vi "GetUserModePrefPath.vi"(8 "error in (no error)":errorcluster) -> (3 "prefpath":path)   [LabVIEW 2023]
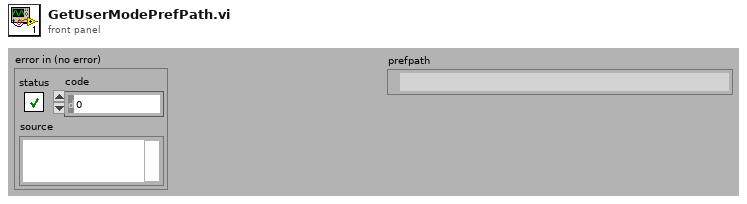
[diagram p1: front panel]
types:
  T1 = enum32{"invalid CPU target", "Motorola 68K", "PowerPC", "Intel x86", "SPARC", "PA-RISC", "MIPS", "Alpha", "ARM", "AMD/Intel x64", "ARM64"}
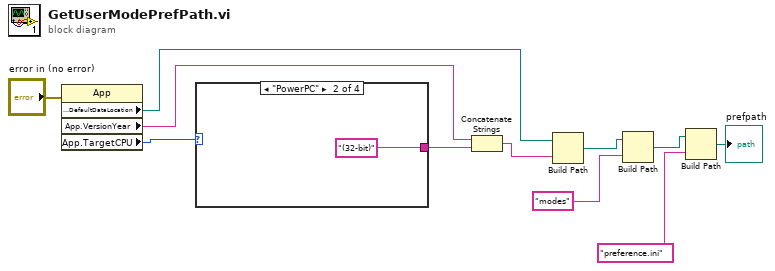
[diagram p0: block diagram]
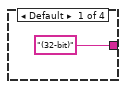
[diagram p2: hidden frame]
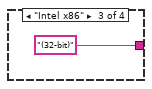
[diagram p3: hidden frame]
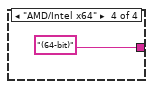
[diagram p4: hidden frame]
diagram:
  n1 = property class="App"(error in="error in (no error)") -> ("App.DefaultDataLocation"=w8:path, "App.VersionYear"=w9:string, "App.TargetCPU"=w11:T1)  [unwired: 1 in, 2 out]
  n2 = case shown="\"PowerPC\"" w11 {
    tunnel: ["(32-bit)" ("string") "(32-bit)" ("string") "(32-bit)" ("string") "(64-bit)" ("string")] -> w10
    frame Default {
    }
    frame "PowerPC" {
    }
    frame "Intel x86" {
    }
    frame "AMD/Intel x64" {
    }
  }
  n3 = Concatenate Strings(w9, w10) -> (w7:string)
  n4 = Build Path(base path=w8, name or relative path=w7) -> (appended path=w6:path)
  n5 = Build Path(base path=w6, name or relative path="modes") -> (appended path=w4:path)
  n6 = Build Path(base path=w4, name or relative path="preference.ini") -> (appended path=→"prefpath":path)
